vi "Test_Flow.vi"() -> ()   [LabVIEW 2026]
doc: "Game_Click 흐름 테스트: 클릭 좌표 배열로 설정→게임 진행, 결과 화면 PNG 저장."
panel:
  out "error out":errorcluster
  out "Draws":i32
  out "Score 2":i32
  out "Score 1":i32
  out "History":T1(array[cluster])
  out "Moves":i32
  out "Status Text":string
  out "Status":T2(ring)
  out "Settings":i32[](array[numeric])
  out "Screen":enum16{"Settings", "Game"}(ring)
  in  "PNG Path":path
  in  "Click Y":i32[](array[numeric])=[635]
  in  "Click X":i32[](array[numeric])=[296]
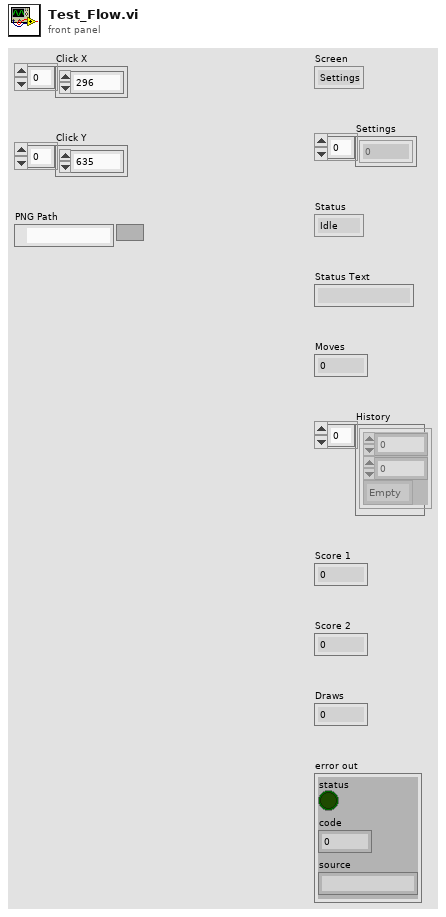
[diagram p1: front panel]
types:
  T1 = cluster{"Row":i32, "Col":i32, "Stone":enum8{"Empty", "Black", "White"}}[]
  T2 = enum16{"Idle", "Player Turn", "AI Thinking", "Game Over"}
  T3 = cluster{"left":i16, "top":i16, "right":i16, "bottom":i16}
  T4 = cluster{"Screen":enum16{"Settings", "Game"}, "Settings":i32[], "Board":cluster{"Grid":enum8{"Empty", "Black", "White"}[][], "Move History":cluster{"Row":i32, "Col":i32, "Stone":enum8{"Empty", "Black", "White"}}[], "Last Move":cluster{"Row":i32, "Col":i32, "Stone":enum8{"Empty", "Black", "White"}}}, "Status":enum16{"Idle", "Player Turn", "AI Thinking", "Game Over"}, "Game ID":u32, "Player Stone":enum8{"Empty", "Black", "White"}, "Hover":cluster{"Row":i32, "Col":i32, "Stone":enum8{"Empty", "Black", "White"}}, "Hover Button":i32, "Win Line":cluster{"Row":i32, "Col":i32, "Stone":enum8{"Empty", "Black", "White"}}[], "Score 1":i32, "Score 2":i32, "Draws":i32, "Status Text":string, "Status Color":u32}
  T5 = cluster{"Grid":enum8{"Empty", "Black", "White"}[][], "Move History":cluster{"Row":i32, "Col":i32, "Stone":enum8{"Empty", "Black", "White"}}[], "Last Move":cluster{"Row":i32, "Col":i32, "Stone":enum8{"Empty", "Black", "White"}}}
  T6 = cluster{"Row":i32, "Col":i32, "Stone":enum8{"Empty", "Black", "White"}}
  T7 = typedef "imagedata.ctl" = cluster{"image type":i32, "image depth":i32, "image":u8[], "mask":u8[], "colors":u32[], "Rectangle":cluster{"left":i16, "top":i16, "right":i16, "bottom":i16}}
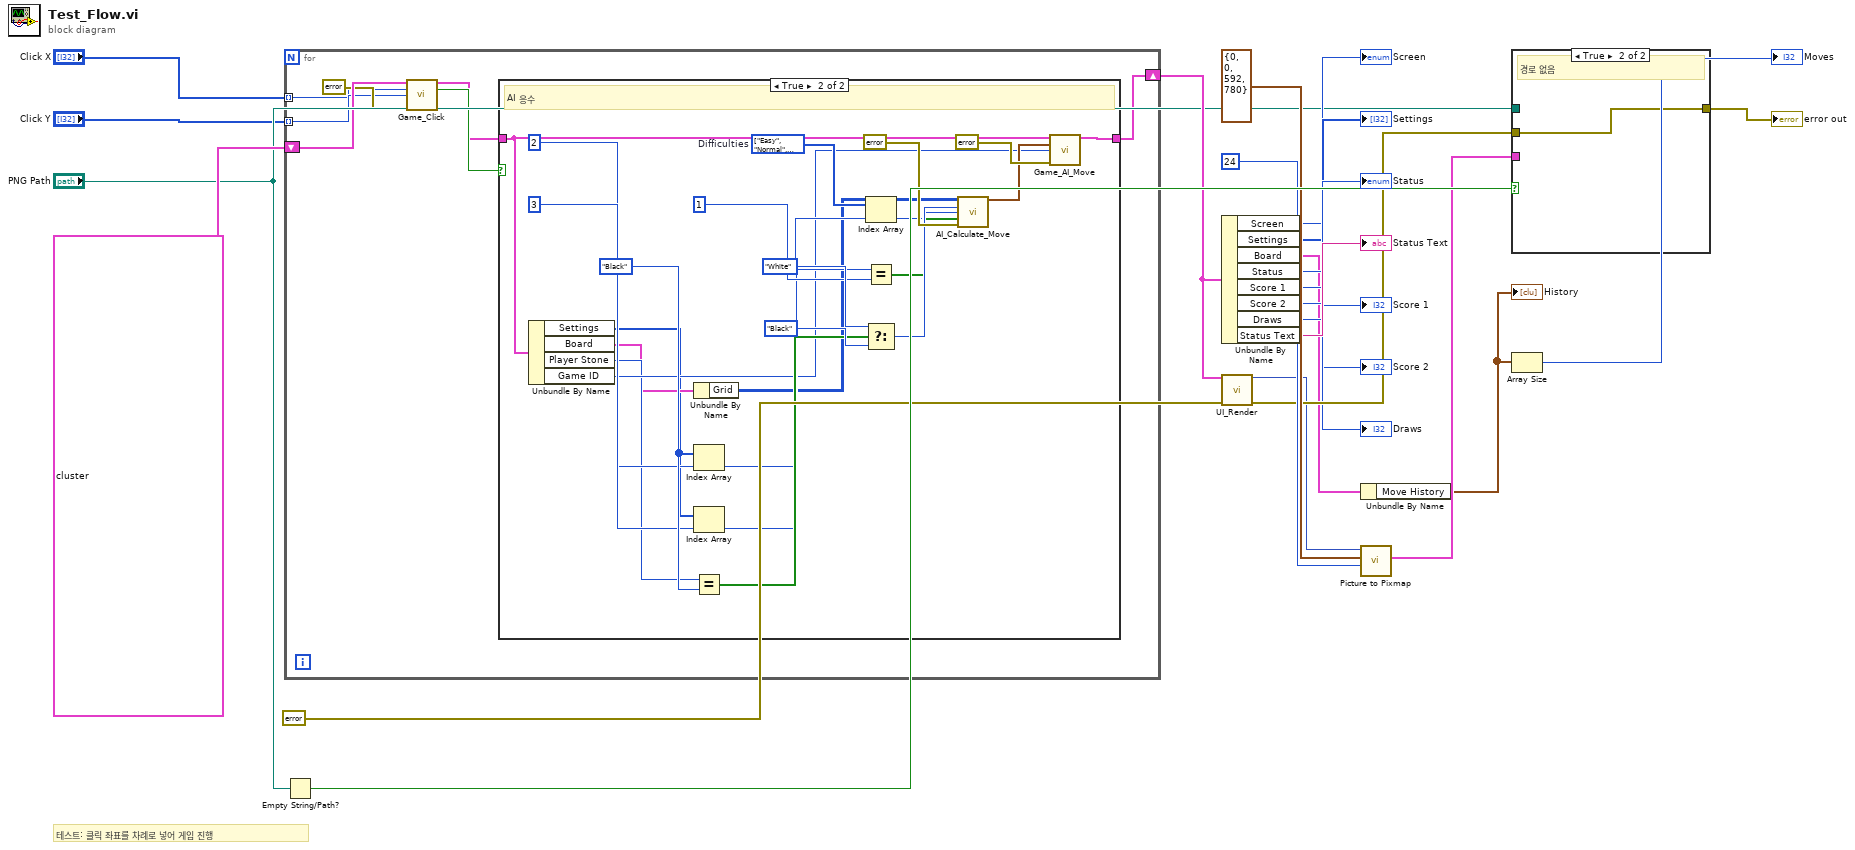
[diagram p0: block diagram]
diagram:
  # "테스트: 클릭 좌표를 차례로 넣어 게임 진행"
  n1 = for {
    tunnel: "Click X" -> [w24] mode=indexing
    tunnel: "Click Y" -> [w25] mode=indexing
    shift-right: [w30] -> w5
    shift-left: T4 {"Screen"=enum."Settings", "Settings"=[0, 0, 1, 1], "Board"={"Grid"=array15x15[225 elements], "Move History"=[], "Last Move"={"Row"=-1, "Col"=-1, "Stone"=enum."Empty"}}, "Status"=enum."Idle", "Game ID"=0, "Player Stone"=enum."Black", "Hover"={"Row"=-1, "Col"=-1, "Stone"=enum."Empty"}, "Hover Button"=-1, "Win Line"=[], "Score 1"=0, "Score 2"=0, "Draws"=0, "Status Text"="", "Status Color"=0} -> [w29]
    n2 = call "Game_Click.vi"("Context"=w29, "X"=w24, "Y"=w25, "error in"=errorcluster {"status"=FALSE, "code"=0, "source"=""}) -> ("Context out"=w27:T4, "Need AI"=w28:bool)  [unwired: 9 in, 1 out]
    n3 = case shown="True" w28 {
      tunnel: w27 -> [w31 w32]
      tunnel: [w31 w54] -> w30
      frame False {
      }
      frame True {
        w38 = enum8{"Easy", "Normal", "Hard", "Master"}[] [enum."Easy", enum."Normal", enum."Hard", enum."Master"] items=["Easy", "Normal", "Hard", "Master"]  # Difficulties
        # "AI 응수"
        n4 = Unbundle By Name(w32) -> ("Settings"=w33:i32[], "Board"=w34:T5, "Player Stone"=w35:enum8{"Empty", "Black", "White"}, "Game ID"=w36:u32)
        n5 = Unbundle By Name(w34) -> ("Grid"=w37:enum8{"Empty", "Black", "White"}[][])
        n6 = Index Array(array=w33, index=2) -> (element=w40:i32)
        n7 = Index Array(array=w33, index=3) -> (element=w43:i32)
        n8 = Equal?(x=w35, y=enum8{"Empty", "Black", "White"}."Black") -> (x = y?=w47:bool[])
        n9 = Index Array(array=w38, index=w40) -> (element=w41:enum8{"Easy", "Normal", "Hard", "Master"})
        n10 = Equal?(x=w43, y=1) -> (x = y?=w45:bool[])
        n11 = Select(t=enum8{"Empty", "Black", "White"}."White", s=w47, f=enum8{"Empty", "Black", "White"}."Black") -> (s? t:f=w50:enum8{"Empty", "Black", "White"})
        n12 = call "AI_Calculate_Move.vi"("Grid"=w37, "AI Stone"=w50, "Difficulty"=w41, "Renju"=w45, "error in"=errorcluster {"status"=FALSE, "code"=0, "source"=""}) -> ("Move"=w52:T6)  [unwired: 7 in, 3 out]
        n13 = call "Game_AI_Move.vi"("Context"=w32, "Move"=w52, "Game ID"=w36, "error in"=errorcluster {"status"=FALSE, "code"=0, "source"=""}) -> ("Context out"=w54:T4)  [unwired: 10 in, 1 out]
      }
    }
  }
  n14 = Empty String/Path?(string/path="PNG Path") -> (empty?=w22:bool)
  n15 = Unbundle By Name(w5) -> ("Screen"=→"Screen":enum16{"Settings", "Game"}, "Settings"=→"Settings":i32[], "Board"=w8:T5, "Status"=→"Status":T2, "Score 1"=→"Score 1":i32, "Score 2"=→"Score 2":i32, "Draws"=→"Draws":i32, "Status Text"=→"Status Text":string)
  n16 = call "UI_Render.vi"("Context"=w5, "error in"=errorcluster {"status"=FALSE, "code"=0, "source"=""}) -> ("Picture"=w17:picture, "error out"=w18:errorcluster)  [unwired: 12 in]
  n17 = Unbundle By Name(w8) -> ("Move History"=w14:T1)
  "History" <- w14
  n18 = call <vilib>:"Picture to Pixmap.vi"("depth"=24, "rect"=T3 {"left"=0, "top"=0, "right"=592, "bottom"=780}, "picture"=w17) -> ("image data"=w21:T7)  [unwired: 7 in, 1 out]
  n19 = case shown="True" w22 {
    tunnel: "PNG Path" -> [w56 _]
    tunnel: w18 -> [w55 w59]
    tunnel: w21 -> [w57 _]
    tunnel: [w58 w59] -> w23
    frame False {
      # "PNG 저장"
      n20 = call <vilib>:"Write PNG File.vi"("error in (no error)"=w55, "image data"=w57, "path to PNG file"=w56) -> ("error out"=w58:errorcluster)  [unwired: 7 in, 1 out]
    }
    frame True {
      # "경로 없음"
    }
  }
  "error out" <- w23
  n21 = Array Size(array=w14) -> (size(s)=→"Moves":i32)
